vi "Error_Popup.vi"(11 "Error In":errorcluster) -> (4 "Stop?":bool, 15 "Error Out":errorcluster)   [LabVIEW 2026, in "Core.lvlib"]
doc: "Error Popup message including the error code, an the source of the error. The user has the option to continue execution of the program, or to stop execution of the program."
uses:
  Core.lvlib
  TypeDefs/Enum_Event_Options.ctl
  TypeDefs/Enum_Events.ctl
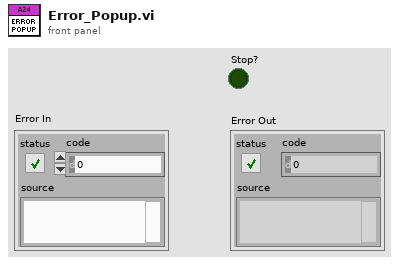
[diagram p1: front panel]
types:
  T1 = typedef "Core.lvlib/Enum_Events.ctl" = enum16{"Stop All", "Stop SubVI", "Update Object"}
  T2 = typedef "Core.lvlib/Enum_Event_Options.ctl" = enum16{"Create", "Generate", "Event Ref", "Destroy"}
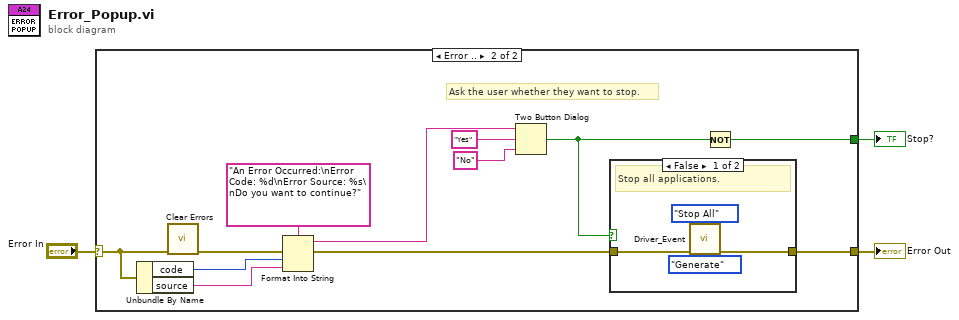
[diagram p0: block diagram]
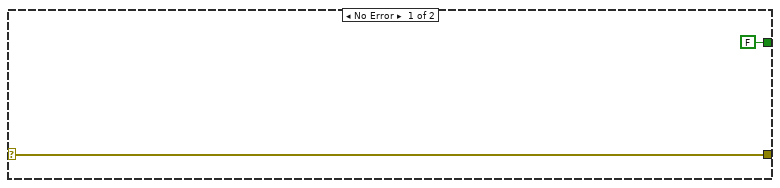
[diagram p2: hidden frame]
diagram:
  n1 = case shown="Error .." "Error In" {
    selector: "Error In" -> [w5 w10]
    tunnel: [w5 w6] -> w3
    tunnel: [FALSE w15] -> w1
    frame No Error {
    }
    frame Error {
      # "Ask the user whether they want to stop."
      n2 = Unbundle By Name(w10) -> ("code"=w13:i32, "source"=w12:string)
      n3 = call <vilib>:"Clear Errors.vi"("error in (no error)"=w10) -> ("error out"=w9:errorcluster)  [unwired: 5 in, 1 out]
      n4 = Format Into String(format string="An Error Occurred:\nError Code: %d\nError Source: %s\nDo you want to continue?", error in=w9, w13, w12) -> (resulting string=w11:string, error out=w8:errorcluster)  [unwired: 1 in]
      n5 = Two Button Dialog(message=w11, 1:"No" ("F button name (\"Cancel\")"), 2:"Yes" ("T button name (\"OK\")")) -> (T button?=w7:bool)
      n6 = case shown="False" w7 {
        tunnel: w8 -> [w21 w22]
        tunnel: [w20 w22] -> w6
        frame False {
          # "Stop all applications."
          n7 = call "Driver_Event.vi"("Event"=Enum_Events."Stop All", "Error In"=w21, "Event Operation"=Enum_Event_Options."Generate") -> ("Error Out"=w20:errorcluster)  [unwired: 11 in, 1 out]
        }
        frame True {
          # "Continue."
        }
      }
      n8 = Not(x=w7) -> (.not. x?=w15:bool)
    }
  }
  "Stop?" <- w1
  "Error Out" <- w3
